vi "AlliGator Panel Storage.vi"(6 "Action (init, dock, undock)":string, 8 "error in (no error)":errorcluster, 9 "Subpanel":string, 11 "Subpanel Paths":path[](array[path])) -> (0 "error out":errorcluster, 1 "Selected Panel":i32, 2 "VI Refnum":refnum<vi>, 3 "Docked Panel List":string[](array[string]), 4 "Image Histogram":i32)   [LabVIEW 2021, in "AlliGator GUI.lvlib"]
uses:
  AlliGator GUI.lvlib
  <userlib>/_OpenG.lib/array/array.llb/Sort 1D Array (String)__ogtk.vi
  <userlib>/_OpenG.lib/array/array.llb/Reorder 1D Array2 (Variant)__ogtk.vi
  <vilib>/Utility/error.llb/Error Cluster From Error Code.vi
  <vilib>/ErrorRing/Error Ring.xnode
  <userlib>/_OpenG.lib/array/array.llb/openg_array.lvlib
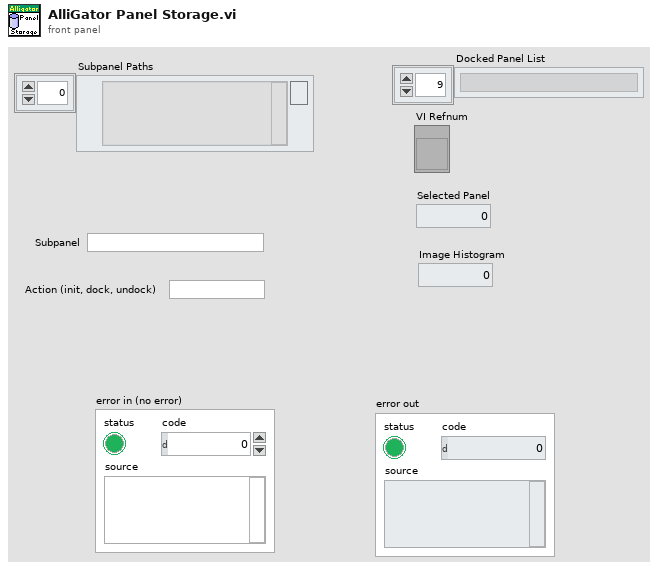
[diagram p1: front panel]
types:
  T1 = enum32{"Invalid", "Standard", "Closed", "Hidden", "Minimized", "Maximized"}
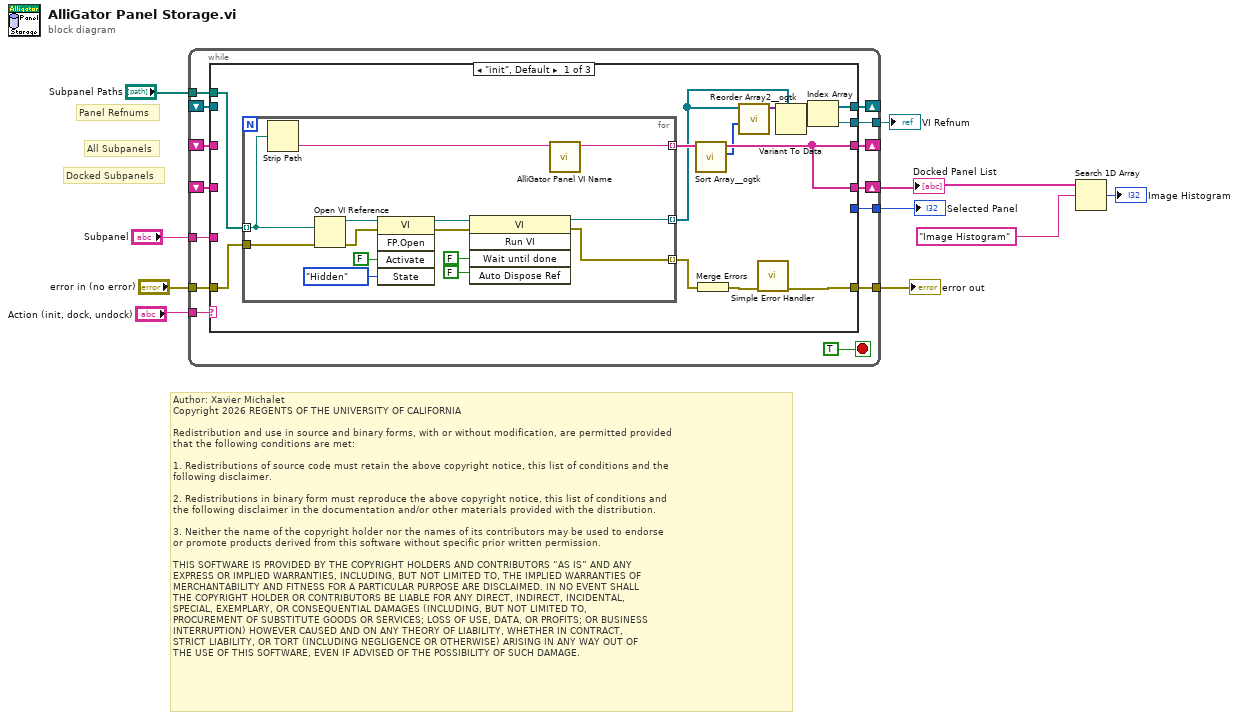
[diagram p0: block diagram]
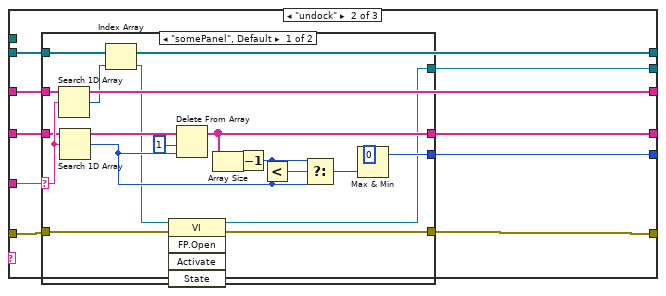
[diagram p2: hidden frame]
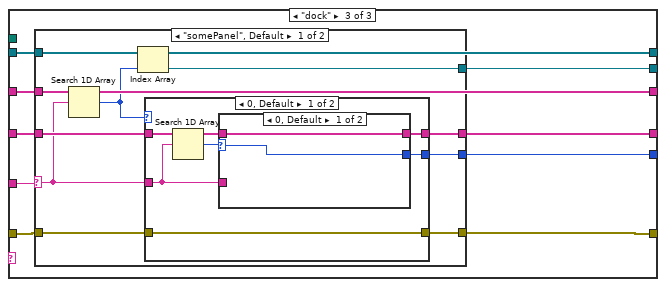
[diagram p4: hidden frame]
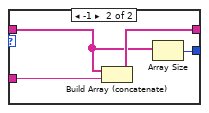
[diagram p5: hidden frame]
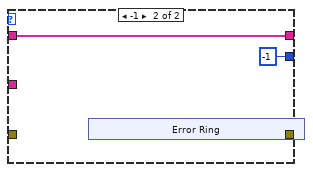
[diagram p6: hidden frame]
diagram:
  # "Panel Refnums"
  # "Docked Subpanels"
  # "All Subpanels"
  # "Author: Xavier Michalet\nCopyright 2026 REGENTS OF THE UNIVERSITY OF CALIFORNIA\n\nRedistribution and use in source and binary forms, with or without modification, are permitted provided\nthat the following conditions are met:\n\n1. Redistributions of source code must retain the above copyright notice, this list of conditions and the\nfollowing disclaimer.\n\n2. Redistributions in binary form must reproduce the above copyright notice, this list of conditions and\nthe following disclaimer in the documentation and/or other materials provided with the distribution.\n\n3. Neither the name of the copyright holder nor the names of its contributors may be used to endorse \nor promote products derived from this software without specific prior written permission.\n\nTHIS SOFTWARE IS PROVIDED BY THE COPYRIGHT HOLDERS AND CONTRIBUTORS “AS IS” AND ANY \nEXPRESS OR IMPLIED WARRANTIES, INCLUDING, BUT NOT LIMITED TO, THE IMPLIED WARRANTIES OF\nMERCHANTABILITY AND FITNESS FOR A PARTICULAR PURPOSE ARE DISCLAIMED. IN NO EVENT SHALL\nTHE COPYRIGHT HOLDER OR CONTRIBUTORS BE LIABLE FOR ANY DIRECT, INDIRECT, INCIDENTAL, \nSPECIAL, EXEMPLARY, OR CONSEQUENTIAL DAMAGES (INCLUDING, BUT NOT LIMITED TO, \nPROCUREMENT OF SUBSTITUTE GOODS OR SERVICES; LOSS OF USE, DATA, OR PROFITS; OR BUSINESS\nINTERRUPTION) HOWEVER CAUSED AND ON ANY THEORY OF LIABILITY, WHETHER IN CONTRACT, \nSTRICT LIABILITY, OR TORT (INCLUDING NEGLIGENCE OR OTHERWISE) ARISING IN ANY WAY OUT OF\nTHE USE OF THIS SOFTWARE, EVEN IF ADVISED OF THE POSSIBILITY OF SUCH DAMAGE."
  n1 = while {
    tunnel: "Subpanel" -> [w24]
    tunnel: "error in (no error)" -> [w23]
    tunnel: "Subpanel Paths" -> [w22]
    shift-right: [w20] -> _
    shift-left: _ -> [w13]
    shift-right: [w19] -> _
    shift-left: _ -> [w14]
    tunnel: "Action (init, dock, undock)" -> [w18]
    tunnel: [w17] -> w6
    shift-right: [w16] -> w3
    shift-left: _ -> [w15]
    tunnel: [w12] -> w5
    tunnel: [w11] -> w4
    stop <- TRUE stop-if-true
    n2 = case shown="\"init\", Default" w18 {
      tunnel: w24 -> [_ w59 w83]
      tunnel: w15 -> [_ w58 w84]
      tunnel: w23 -> [w34 w57 w85]
      tunnel: w22 -> [w35 _ _]
      tunnel: [w27 w53 w87] -> w20
      tunnel: [w30 w54 w88] -> w19
      tunnel: [w25 w56 w86] -> w17
      tunnel: [w30 w55 w82] -> w16
      tunnel: w14 -> [_ w54 w88]
      tunnel: w13 -> [_ w53 w87]
      tunnel: [_ w52 w80] -> w12
      tunnel: [w36 w51 w81] -> w11
      frame "init", Default {
        n3 = for {
          tunnel: w35 -> [w39] mode=indexing
          tunnel: w34 -> [w41]
          tunnel: [w50] -> w31 mode=indexing
          tunnel: [w37] -> w33 mode=indexing
          tunnel: [w38] -> w26 mode=indexing
          n4 = Strip Path(path=w39) -> (name=w40:string)  [unwired: 1 out]
          n5 = Open VI Reference(vi path=w39, error in (no error)=w41) -> (vi reference=w44:refnum<vi>, error out=w45:errorcluster)  [unwired: 4 in]
          n6 = invoke class="VI" method="FP.Open"(reference=w44, error in=w45, "Activate"=FALSE ("Activate?"), "State"=T1."Hidden") -> (reference out=w48:refnum<vi>, error out=w49:errorcluster)  [unwired: 1 in, 3 out]
          n7 = invoke class="VI" method="Run VI"(reference=w48, error in=w49, "Wait until done"=FALSE, "Auto Dispose Ref"=FALSE) -> (reference out=w38:refnum<vi>, error out=w37:errorcluster)  [unwired: 1 in, 3 out]
          n8 = call "AlliGator Panel VI Name.vi"("Panel VI Name"=w40) -> ("Panel Name"=w50:string)  [unwired: 10 in]
        }
        n9 = call-poly <userlib>:"Sort Array__ogtk.vi"("Array in"=w31) -> ("Sorted Pointers"=w29:i32[], "Sorted Array out"=w30:string[])  [unwired: 9 in]
        n10 = Merge Errors(w33) -> (w32:errorcluster)
        n11 = call-poly <userlib>:"Reorder Array2__ogtk.vi"("indices"=w29, "array"=w26) -> ("reordered array"=w28:variant[])  [unwired: 9 in]
        n12 = call <vilib>:"Simple Error Handler.vi"("error in (no error)"=w32) -> ("error out"=w25:errorcluster)  [unwired: 4 in, 4 out]
        n13 = Variant To Data(type=w26, Variant=w28) -> (data=w27:refnum<vi>[])  [unwired: 1 in, 1 out]
        n14 = Index Array(array=w27) -> (element=w36:refnum<vi>)  [unwired: 1 in]
      }
      frame "undock" {
        n15 = case shown="\"somePanel\", Default" w59 {
          selector: w59 -> [w76 _]
          tunnel: w58 -> [w75 w79]
          tunnel: w57 -> [w70 w78]
          tunnel: [w65 w78] -> w56
          tunnel: [w64 w79] -> w55
          tunnel: w54 -> [w63 _]
          tunnel: w53 -> [w62 _]
          tunnel: [w61 _] -> w52
          tunnel: [w60 _] -> w51
          frame "somePanel", Default {
            n16 = Search 1D Array(1D array=w63, element=w76) -> (index of element=w67:i32)  [unwired: 1 in]
            n17 = Search 1D Array(1D array=w75, element=w76) -> (index of element=w77:i32)  [unwired: 1 in]
            n18 = Index Array(array=w62, index=w67) -> (element=w69:refnum<vi>)
            n19 = invoke class="VI" method="FP.Open"(reference=w69, error in=w70) -> (reference out=w60:refnum<vi>, error out=w65:errorcluster)  [unwired: 3 in, 3 out]
            n20 = Delete From Array(array=w75, length=1, index=w77) -> (array with subset deleted=w64:string[])  [unwired: 1 out]
            n21 = Array Size(array=w64) -> (size(s)=w71:i32)
            n22 = Decrement(x=w71) -> (x-1=w73:i32)
            n23 = Less?(x=w73, y=w77) -> (x < y?=w72:bool)
            n24 = Select(t=w73, s=w72, f=w77) -> (s? t:f=w74:i32)
            n25 = Max & Min(x=0, y=w74) -> (max(x,y)=w61:i32)  [unwired: 1 out]
          }
          frame "" {
          }
        }
      }
      frame "dock" {
        n26 = case shown="\"somePanel\", Default" w83 {
          selector: w83 -> [w92 _]
          tunnel: w88 -> [w98 _]
          tunnel: w87 -> [w97 _]
          tunnel: [w95 w118] -> w86
          tunnel: w85 -> [w94 w118]
          tunnel: w84 -> [w93 w119]
          tunnel: [w91 w119] -> w82
          tunnel: [w90 _] -> w81
          tunnel: [w89 _] -> w80
          frame "somePanel", Default {
            n27 = Search 1D Array(1D array=w98, element=w92) -> (index of element=w96:i32)  [unwired: 1 in]
            n28 = Index Array(array=w97, index=w96) -> (element=w90:refnum<vi>)
            n29 = case shown="0, Default" w96 {
              tunnel: [w104 w113] -> w95
              tunnel: w94 -> [w104 _]
              tunnel: w93 -> [w101 w112]
              tunnel: w92 -> [w100 _]
              tunnel: [w103 w112] -> w91
              tunnel: [w102 -1] -> w89
              frame 0, Default {
                n30 = Search 1D Array(1D array=w101, element=w100) -> (index of element=w99:i32)  [unwired: 1 in]
                n31 = case shown="0, Default" w99 {
                  selector: w99 -> [w106 _]
                  tunnel: w100 -> [_ w110]
                  tunnel: [w105 w109] -> w103
                  tunnel: w101 -> [w105 w108]
                  tunnel: [w106 w107] -> w102
                  frame 0, Default {
                  }
                  frame -1 {
                    n32 = Build Array (concatenate)(w108, w110) -> (w109:string[])
                    n33 = Array Size(array=w108) -> (size(s)=w107:i32)
                  }
                }
              }
              frame -1 {
                n34 = xnode "Error Ring"() -> ("error out"=w113:errorcluster)
              }
            }
          }
          frame "" {
          }
        }
      }
    }
  }
  "Docked Panel List" <- w3
  "error out" <- w6
  "Selected Panel" <- w5
  "VI Refnum" <- w4
  n35 = Search 1D Array(1D array=w3, element="Image Histogram") -> (index of element=→"Image Histogram":i32)  [unwired: 1 in]
